vi "VIH - CHM Project - Add External HTML Files to Project File Paths.vi"(10 "Extra HTML files":path[](array[path]), 11 "Project Files":T2) -> (3 "Project Files out":T2)   [LabVIEW 2014]
doc: "::: VI Helpeks :::\nCopyright (c) 2000-2026 Konstantin Shifershteyn. All rights reserved."
uses:
  _VIH HelpGen - Palette.llb/VIH HelpGen Typedef - Palette - Item Type Enum.ctl
panel:
  # "VI Helpeks\nCopyright (c) 2012-2026 Konstantin Shifershteyn"
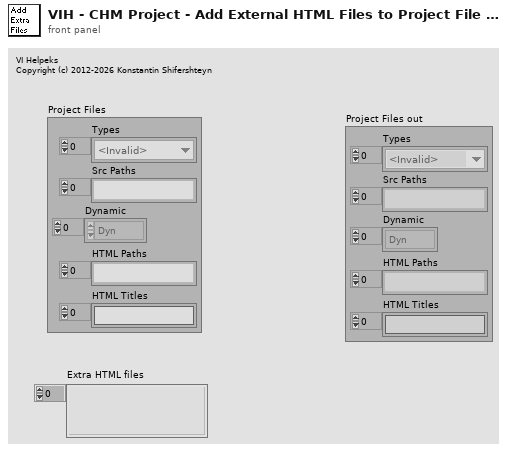
[diagram p1: front panel]
types:
  T1 = typedef "VIH HelpGen Typedef - Palette - Item Type Enum.ctl" = enum32{"<Invalid>", "<unknown>", "VI", "Menu", "LV Func", "Express VI", "Poly VI", "CTL", "HTML"}
  T2 = cluster{"Types":T1[], "Src Paths":path[], "Dynamic":enum16{"Dyn", "Stat", "Both"}[], "HTML Paths":path[], "HTML Titles":string[]}
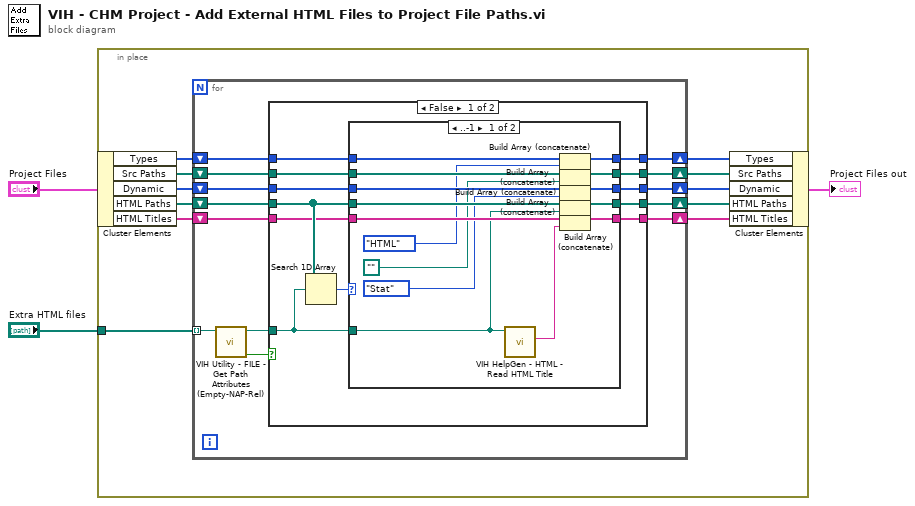
[diagram p0: block diagram]
diagram:
  n1 = in-place {
    in-place-border: "Extra HTML files" -> [w14]
    n2 = in-place-cluster #1("Project Files") -> ("Types"=w13:T1[], "Src Paths"=w12:path[], "Dynamic"=w11:enum16{"Dyn", "Stat", "Both"}[], "HTML Paths"=w10:path[], "HTML Titles"=w9:string[])
    n3 = for {
      shift-right: [w19] -> w4
      shift-left: w9 -> [w18]
      shift-right: [w21] -> w5
      shift-left: w10 -> [w20]
      shift-right: [w23] -> w6
      shift-left: w11 -> [w22]
      shift-right: [w25] -> w7
      shift-left: w12 -> [w24]
      shift-right: [w27] -> w8
      shift-left: w13 -> [w26]
      tunnel: w14 -> [w17] mode=indexing
      n4 = call "VIH Utility - FILE - Get Path Attributes (Empty-NAP-Rel).vi"("Path"=w17) -> ("Not A Path or Empty path"=w15:bool, "dup Path"=w16:path)  [unwired: 6 in, 3 out]
      n5 = case shown="False" w15 {
        tunnel: [w38 w64] -> w27
        tunnel: w26 -> [w37 w64]
        tunnel: [w36 w63] -> w25
        tunnel: w24 -> [w35 w63]
        tunnel: [w34 w62] -> w23
        tunnel: w22 -> [w33 w62]
        tunnel: [w32 w61] -> w21
        tunnel: w20 -> [w31 w61]
        tunnel: [w30 w60] -> w19
        tunnel: w18 -> [w29 w60]
        tunnel: w16 -> [w28 _]
        frame False {
          n6 = Search 1D Array(1D array=w31, element=w28) -> (index of element=w39:i32)  [unwired: 1 in]
          n7 = case shown="..-1" w39 {
            tunnel: [w53 w59] -> w38
            tunnel: w37 -> [w54 w59]
            tunnel: [w48 w58] -> w36
            tunnel: w35 -> [w52 w58]
            tunnel: [w47 w57] -> w34
            tunnel: w33 -> [w51 w57]
            tunnel: [w46 w56] -> w32
            tunnel: w31 -> [w50 w56]
            tunnel: [w45 w55] -> w30
            tunnel: w29 -> [w49 w55]
            tunnel: w28 -> [w44 _]
            frame ..-1 {
              n8 = call "VIH HelpGen - HTML - Read HTML Title.vi"("HTML File Path"=w44) -> ("Title"=w43:string)  [unwired: 8 in, 2 out]
              n9 = Build Array (concatenate)(w54, VIH_HelpGen_Typedef_-_Palette_-_Item_Type_Enum."HTML" ("Item/File Type")) -> (w53:T1[])
              n10 = Build Array (concatenate)(w52, path "") -> (w48:path[])
              n11 = Build Array (concatenate)(w51, enum16{"Dyn", "Stat", "Both"}."Stat") -> (w47:enum16{"Dyn", "Stat", "Both"}[])
              n12 = Build Array (concatenate)(w50, w44) -> (w46:path[])
              n13 = Build Array (concatenate)(w49, w43) -> (w45:string[])
            }
            frame 0.. {
            }
          }
        }
        frame True {
        }
      }
    }
    n14 = in-place-cluster #1("Types"=w8, "Src Paths"=w7, "Dynamic"=w6, "HTML Paths"=w5, "HTML Titles"=w4) -> (→"Project Files out":T2)
  }
